vi "bcrypt BCryptGenRandom.vi"(0 "byte count":u32=16, 5 "hAlgorithm":u64, 7 "dwFlags":u32=2, 11 "error in":errorcluster) -> (4 "random bytes":u8[](array[numeric]), 6 "return value":i32, 15 "error out":errorcluster)   [LabVIEW 2020, in "RemoteVI.lvlib"]
doc: "Fills byte count bytes with cryptographically secure random numbers through bcrypt.dll BCryptGenRandom (stdcall, called in any thread) with the system-preferred random number generator (hAlgorithm NULL, dwFlags BCRYPT_USE_SYSTEM_PREFERRED_RNG = 2). return value is the NTSTATUS: 0 on success. When error in carries an error the DLL is not called. Generated by scripts\\Build Win32 Wrappers.vi - do not edit by hand, rebuild it."
uses:
  RemoteVI.lvlib
  bcrypt.dll
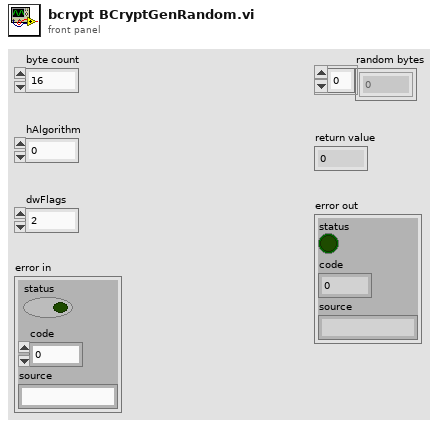
[diagram p1: front panel]
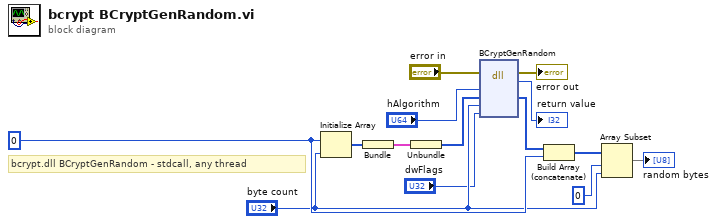
[diagram p0: block diagram]
diagram:
  w10 = u8 0
  # "bcrypt.dll BCryptGenRandom - stdcall, any thread"
  n1 = Initialize Array(w10, "byte count") -> (w12:u8[])
  n2 = Bundle(w12) -> (w13:cluster{u8[]})  [unwired: 1 in]
  n3 = Unbundle(w13) -> (w3:u8[])
  n4 = dll-call lib="bcrypt.dll" fn="BCryptGenRandom"(error in="error in", "hAlgorithm"="hAlgorithm", "pbBuffer"=w3, "cbBuffer"="byte count", "dwFlags"="dwFlags") -> (error out=→"error out":errorcluster, →"return value":i32, "pbBuffer"=w2:u8[])  [unwired: 5 in, 1 out]
  n5 = Build Array (concatenate)(w2, w10) -> (w14:u8[])
  n6 = Array Subset(array=w14, index=0, length="byte count") -> (→"random bytes":u8[])
